vi "DSS-test-param_tables.vi"(8 "error in":errorcluster) -> (0 "error out":errorcluster)   [LabVIEW 2020, in "DSS-Tests.lvlib"]
doc: "Caraya test of RDC-water- and RDC-saltwater-generate_perm_param_to_share, run by VI Server from -5 to 60 C in 0.1 C steps: every field of every row of the panel-only Array is checked against its golden file."
uses:
  DSS-Tests.lvlib
  <vilib>/addons/_JKI Toolkits/Caraya/classes/Test/Test.lvclass
  <vilib>/addons/_JKI Toolkits/Caraya/classes/Assert/Assert.lvclass
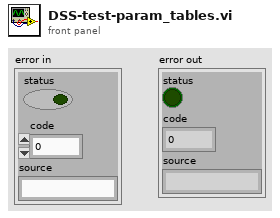
[diagram p1: front panel]
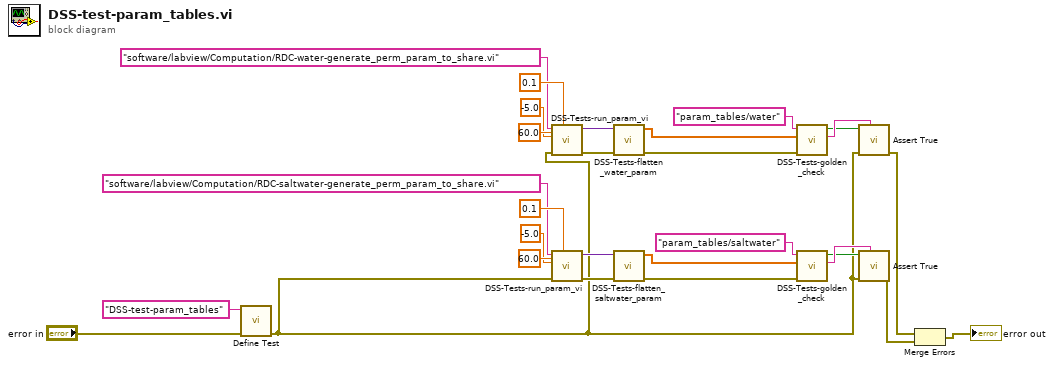
[diagram p0: block diagram]
diagram:
  n1 = call <vilib>:"Define Test.vi"("error in (no error)"="error in", "Label (VI Title)"="DSS-test-param_tables") -> ("error out"=w3:errorcluster)  [unwired: 8 in, 1 out]
  n2 = call "DSS-Tests-run_param_vi.vi"("increment temp"=0.1, "error in"=w3, "stop temp"=60.0, "start temp"=-5.0, "vi relative path"="software/labview/Computation/RDC-water-generate_perm_param_to_share.vi") -> ("error out"=w9:errorcluster, "array variant"=w8:variant)  [unwired: 5 in]
  n3 = call "DSS-Tests-run_param_vi.vi"("increment temp"=0.1, "error in"=w3, "stop temp"=60.0, "start temp"=-5.0, "vi relative path"="software/labview/Computation/RDC-saltwater-generate_perm_param_to_share.vi") -> ("error out"=w21:errorcluster, "array variant"=w20:variant)  [unwired: 5 in]
  n4 = call "DSS-Tests-flatten_water_param.vi"("error in"=w9, "array variant"=w8) -> ("error out"=w11:errorcluster, "flat"=w10:dbl[])  [unwired: 8 in]
  n5 = call "DSS-Tests-flatten_saltwater_param.vi"("error in"=w21, "array variant"=w20) -> ("error out"=w23:errorcluster, "flat"=w22:dbl[])  [unwired: 8 in]
  n6 = call "DSS-Tests-golden_check.vi"("error in"=w11, "actual"=w10, "golden name"="param_tables/water") -> ("message"=w14:string, "pass"=w13:bool)  [unwired: 6 in, 1 out]
  n7 = call "DSS-Tests-golden_check.vi"("error in"=w23, "actual"=w22, "golden name"="param_tables/saltwater") -> ("message"=w26:string, "pass"=w25:bool)  [unwired: 6 in, 1 out]
  n8 = call <vilib>:"Assert True.vi"("Label"=w14, "error in (no error)"=w3, "True?"=w13) -> ("error out"=w15:errorcluster)  [unwired: 7 in, 1 out]
  n9 = call <vilib>:"Assert True.vi"("Label"=w26, "error in (no error)"=w3, "True?"=w25) -> ("error out"=w27:errorcluster)  [unwired: 7 in, 1 out]
  n10 = Merge Errors(w15, w27) -> (→"error out":errorcluster)
